vi "FuncVI-viOpenFP.vi"(5 "InstanceRef":T2, 9 "arg list":T1[](array[typedef]) {"num" format="%.2f"}) -> (0 "error out":bool, 3 "result":T1 {"num" format="%.2f"})   [LabVIEW 2021]
doc: "::: CalcExpress Toolkit :::\nCopyright (c) 2000-2026 Konstantin Shifershteyn. All rights reserved."
uses:
  cetypes.llb/CalcExpress Function Argument Info.ctl
  cetypes.llb/CalcExpress Instance RefNum.ctl
panel:
  in  "max arg num":i32=2
  in  "min arg num":i32=1
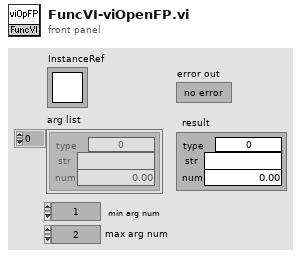
[diagram p1: front panel]
types:
  T1 = typedef "CalcExpress Function Argument Info.ctl" = cluster{"type":u32, "str":string, "num":dbl}
  T2 = typedef "CalcExpress Instance RefNum.ctl" = refnum<k1>
  T3 = enum32{"String", "DBL Number", "identifier", "1D Array of DBL", "2D Array of DBL", "CDB Number", "1D Array of CDB", "2D Array of CDB", "1D Array of String", "2D Array of String", "Unknown data type"}
  T4 = cluster{"index":i32, "data type":enum32{"String", "DBL Number", "identifier", "1D Array of DBL", "2D Array of DBL", "CDB Number", "1D Array of CDB", "2D Array of CDB", "1D Array of String", "2D Array of String", "Unknown data type"}, "default num":dbl, "default str":string}[]
  T5 = enum32{"Invalid", "Standard", "Closed", "Hidden", "Minimized", "Maximized"}
  T6 = cluster{"use this constant to specify a predefined type":enum32{"String", "DBL Number", "identifier", "1D Array of DBL", "2D Array of DBL", "CDB Number", "1D Array of CDB", "2D Array of CDB", "1D Array of String", "2D Array of String", "Unknown data type"}, string, "code":i32}
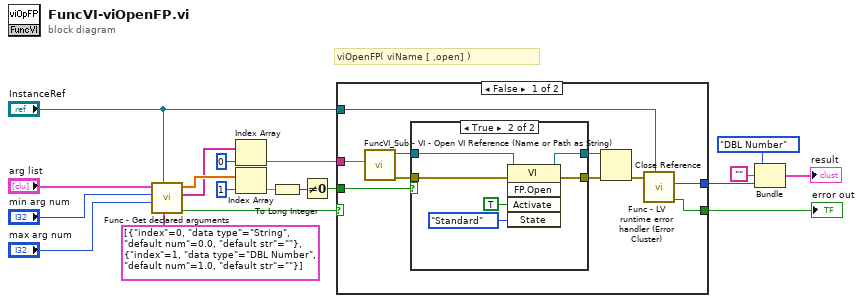
[diagram p0: block diagram]
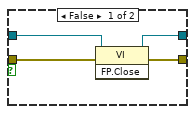
[diagram p2: hidden frame]
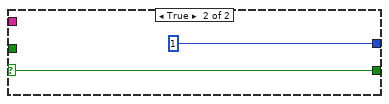
[diagram p3: hidden frame]
diagram:
  # "viOpenFP( viName [ ,open] )"
  n1 = call "Func - Get declared arguments.vi"("arg descriptors"=T4 [{"index"=0, "data type"=enum."String", "default num"=0.0, "default str"=""}, {"index"=1, "data type"=enum."DBL Number", "default num"=1.0, "default str"=""}] ("args descriptors"), "InstanceRef"="InstanceRef", "max arg num"="max arg num", "min arg num"="min arg num", "arg list"="arg list") -> ("error out"=w3:bool, "str list"=w12:string[], "num list"=w13:dbl[])  [unwired: 3 in, 1 out]
  n2 = Index Array(array=w12, index=0) -> (element=w1:string)
  n3 = Index Array(array=w13, index=1) -> (element=w10:dbl)
  n4 = To Long Integer(number=w10) -> (32bit integer=w11:i32)
  n5 = Not Equal To 0?(x=w11) -> (x != 0?=w9:bool)
  n6 = case shown="False" w3 {
    selector: w3 -> [_ w41]
    tunnel: w1 -> [w29 _]
    tunnel: w9 -> [w20 _]
    tunnel: [w22 w41] -> w7
    tunnel: "InstanceRef" -> [w23 _]
    tunnel: [w21 1 ("code")] -> w2
    frame False {
      n7 = call "FuncVI_Sub - VI - Open VI Reference (Name or Path as String).vi"("VI name or path"=w29) -> ("error out"=w28:errorcluster, "VI Refnum"=w27:refnum<vi>)  [unwired: 9 in]
      n8 = case shown="True" w20 {
        tunnel: w28 -> [w33 w38]
        tunnel: w27 -> [w32 w39]
        tunnel: [w30 w36] -> w26
        tunnel: [w31 w37] -> w25
        frame False {
          n9 = invoke class="VI" method="FP.Close"(reference=w32, error in=w33) -> (reference out=w31:refnum<vi>, error out=w30:errorcluster)  [unwired: 1 in, 1 out]
        }
        frame True {
          n10 = invoke class="VI" method="FP.Open"(reference=w39, error in=w38, "Activate"=TRUE ("Activate?"), "State"=T5."Standard") -> (reference out=w37:refnum<vi>, error out=w36:errorcluster)  [unwired: 1 in, 3 out]
        }
      }
      n11 = Close Reference(reference=w25, error in (no error)=w26) -> (error out=w24:errorcluster)
      n12 = call "Func - LV runtime error handler (Error Cluster).vi"("InstanceRef"=w23, "LabVIEW error"=w24) -> ("error out"=w22:bool, "LV error code"=w21:i32)  [unwired: 4 in, 2 out]
    }
    frame True {
    }
  }
  "error out" <- w7
  n13 = Bundle("use this constant to specify a predefined type"=T3."DBL Number", "", "code"=w2) -> (→"result":T6)  [unwired: 1 in]
